vi "Convert Point to Coord.vi"(8 "error in":errorcluster, 10 "Overlay":T1={"Name"="p0", "Data"={"Points"=array[7388 elements], "Voltages"=array[7388 elements]}, "Changes"={"MD5 Digest"="", "Changed?"=FALSE}}, 11 "BigMAQ in":refnum<class "BigMAQ.lvclass">) -> (0 "error out":errorcluster, 1 "Voltage Constant?":bool, 2 "output cluster":T1, 3 "BigMAQ out":refnum<class "BigMAQ.lvclass">)   [LabVIEW 2019, in "BigMAQ.lvclass"]
uses:
  BigMAQ.lvclass
  Overlay.ctl
  BigMAQ.lvclass/BigMAQ.ctl
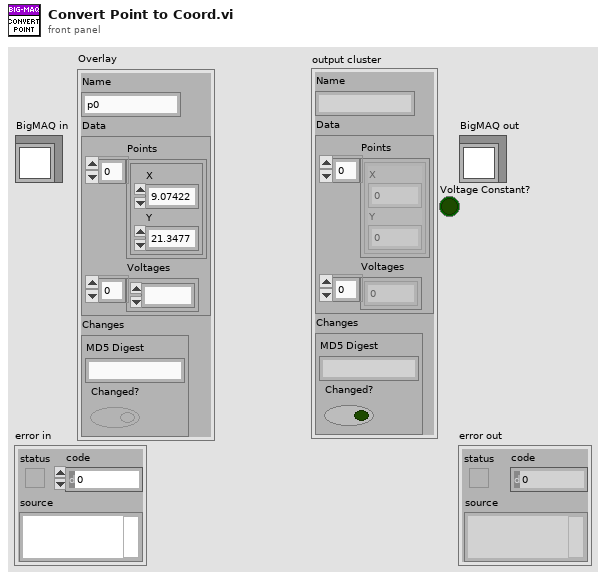
[diagram p1: front panel]
types:
  T1 = typedef "BigMAQ.lvclass/Overlay.ctl" = cluster{"Name":string, "Data":cluster{"Points":cluster{"X":dbl, "Y":dbl}[], "Voltages":dbl[]}, "Changes":cluster{"MD5 Digest":string, "Changed?":bool}}
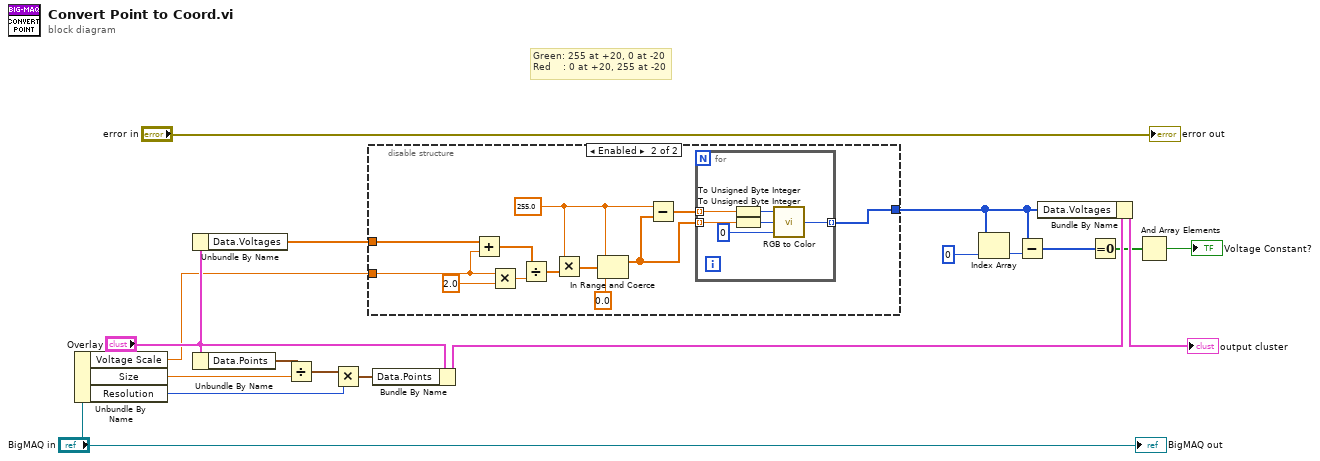
[diagram p0: block diagram]
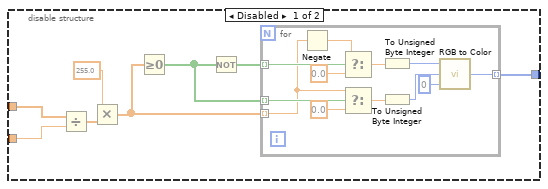
[diagram p2: hidden frame]
diagram:
  # "Green: 255 at +20, 0 at -20\nRed    : 0 at +20, 255 at -20"
  n1 = Unbundle By Name("BigMAQ in") -> ("Voltage Scale"=w1:dbl, "Size"=w4:dbl, "Resolution"=w3:i32)
  n2 = Unbundle By Name("Overlay") -> ("Data.Voltages"=w14:dbl[])
  n3 = Unbundle By Name("Overlay") -> ("Data.Points"=w17:cluster{"X":dbl, "Y":dbl}[])
  n4 = Divide(x=w17, y=w4) -> (x/y=w16:cluster{"X":dbl, "Y":dbl}[])
  n5 = Multiply(x=w16, y=w3) -> (x*y=w15:cluster{"X":dbl, "Y":dbl}[])
  n6 = disable-structure shown="Enabled" {
    disable-tunnel: w14 -> [w26 w41]
    disable-tunnel: [w20 w39] -> w2
    disable-tunnel: w1 -> [w19 w40]
    frame Disabled {
      n7 = Divide(x=w26, y=w19) -> (x/y=w25:dbl[])
      n8 = Multiply(x=255.0, y=w25) -> (x*y=w24:dbl[])
      n9 = Greater Or Equal To 0?(x=w24) -> (x >= 0?=w21:bool[])
      n10 = Not(x=w21) -> (.not. x?=w22:bool[])
      n11 = for {
        tunnel: w22 -> [w38] mode=indexing
        tunnel: w24 -> [w31] mode=indexing
        tunnel: w21 -> [w32] mode=indexing
        tunnel: [w27] -> w20 mode=indexing
        n12 = Negate(x=w31) -> (-x=w34:dbl)
        n13 = Select(t=w34, s=w38, f=0.0) -> (s? t:f=w37:dbl)
        n14 = Select(t=w31, s=w32, f=0.0) -> (s? t:f=w30:dbl)
        n15 = To Unsigned Byte Integer(number=w37) -> (unsigned 8bit integer=w36:u8)
        n16 = To Unsigned Byte Integer(number=w30) -> (unsigned 8bit integer=w29:u8)
        n17 = call <vilib>:"RGB to Color.vi"("B"=u8 0, "G"=w29, "R"=w36) -> ("Color"=w27:u32)
      }
    }
    frame Enabled {
      w42 = 255.0
      n18 = Add(x=w41, y=w40) -> (x+y=w43:dbl[])
      n19 = Multiply(x=w40, y=2.0) -> (x*y=w47:dbl)
      n20 = Divide(x=w43, y=w47) -> (x/y=w50:dbl[])
      n21 = Multiply(x=w42, y=w50) -> (x*y=w49:dbl[])
      n22 = In Range and Coerce(upper limit=w42, x=w49, lower limit=0.0) -> (coerced(x)=w45:dbl[])  [unwired: 1 out]
      n23 = Subtract(x=w42, y=w45) -> (x-y=w44:dbl[])
      n24 = for {
        tunnel: [w53] -> w39 mode=indexing
        tunnel: w45 -> [w52] mode=indexing
        tunnel: w44 -> [w51] mode=indexing
        n25 = To Unsigned Byte Integer(number=w51) -> (unsigned 8bit integer=w56:u8)
        n26 = To Unsigned Byte Integer(number=w52) -> (unsigned 8bit integer=w55:u8)
        n27 = call <vilib>:"RGB to Color.vi"("B"=u8 0, "G"=w55, "R"=w56) -> ("Color"=w53:u32)
      }
    }
  }
  n28 = Bundle By Name(cluster="Overlay", "Data.Points"=w15) -> (w13:T1)
  n29 = Index Array(array=w2, index=0) -> (element=w10:u32)
  n30 = Subtract(x=w2, y=w10) -> (x-y=w9:u32[])
  n31 = Bundle By Name(cluster=w13, "Data.Voltages"=w2) -> (→"output cluster":T1)
  n32 = Equal To 0?(x=w9) -> (x = 0?=w8:bool[])
  n33 = And Array Elements(Boolean array=w8) -> (logical AND=→"Voltage Constant?":bool)
  "error out" <- "error in"
  "BigMAQ out" <- "BigMAQ in"
